vi "http set proxy.vi"(8 "error in (no error)":errorcluster, 11 "proxy server (none)":string="direct") -> (0 "error out":errorcluster)   [LabVIEW 2020, in "reqwest-labview.lvlib"]
uses:
  reqwest-labview.lvlib
  lib_reqwest_labview_64.dll
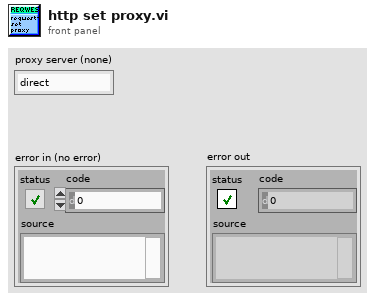
[diagram p1: front panel]
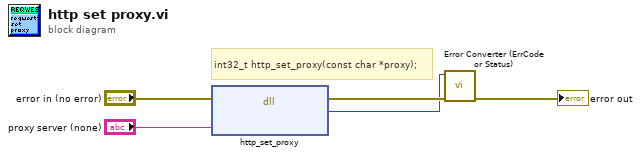
[diagram p0: block diagram]
diagram:
  # "int32_t http_set_proxy(const char *proxy);"
  n1 = dll-call lib="C:/sw/labview-client/submodules/reqwest-labview/lv-src/shared-library/lib_reqwest_labview_*.*" fn="http_set_proxy" ("reqwest_labview_*.*:http_get")(error in="error in (no error)", "proxy"="proxy server (none)") -> (error out=w2:errorcluster, "return type"=w1:i32)  [unwired: 3 in, 1 out]
  n2 = call "Error Converter (ErrCode or Status).vi"("error in (no error)"=w2, "error code"=w1) -> ("error out"=→"error out":errorcluster)  [unwired: 9 in]
